vi "HEALTH_LABVIEW_V8.vi"() -> ()   [LabVIEW 2026]
uses:
  <vilib>/addons/control/pid/pid.llb/PID (DBL).vi
  <vilib>/addons/control/pid/NI_PID_pid.lvlib
panel:
  out "EXT SURF RTD HX SIDE":dbl format="%#_3g"
  out "BLOCK RTD HEATER SIDE":dbl format="%#_3g"
  out "BLOCK RTD HX SIDE":dbl format="%#_3g"
  out "EXT SURF RTD HEATER SIDE":dbl format="%#_3g"
  out "COPPER BLOCK RTDs":cluster{dbl, dbl, dbl, dbl}(graph)
  in  "CLEAR GRAPHS":bool
  in  "PUMP PID GAINS":T1={"proportional gain (Kc)"=1.0, "integral time (Ti, min)"=0.01, "derivative time (Td, min)"=0.0} {"derivative time (Td, min)" format="%.3f"; "integral time (Ti, min)" format="%.3f"; "proportional gain (Kc)" format="%.3f"}
  in  "TARGET FLOW RATE (LPM)":dbl format="%.2f"
  out "OUTLET TEMP (C)":dbl format="%#_3g"
  out "INLET TEMP (C)":dbl format="%#_3g"
  out "PRESSURE DROP (PSI)":dbl(graph)
  out "DELTA T (C)":dbl format="%#_3f"
  out "DELTA T (C)":dbl(graph)
  out "COOLANT FLOW RATE":dbl(graph)
  in  "PUMP ON/OFF":bool
  in  "HEATER ON/OFF":bool
  in  "stop":bool
  out "Error String":string
  out "error out":errorcluster
  out "ConnectionType Out":i32
  out "DeviceType Out":i32
  in  "Identifier":string="LJM_idANY"
  in  "ConnectionType":string="LJM_ctANY"
  in  "DeviceType":string="LJM_dtANY"
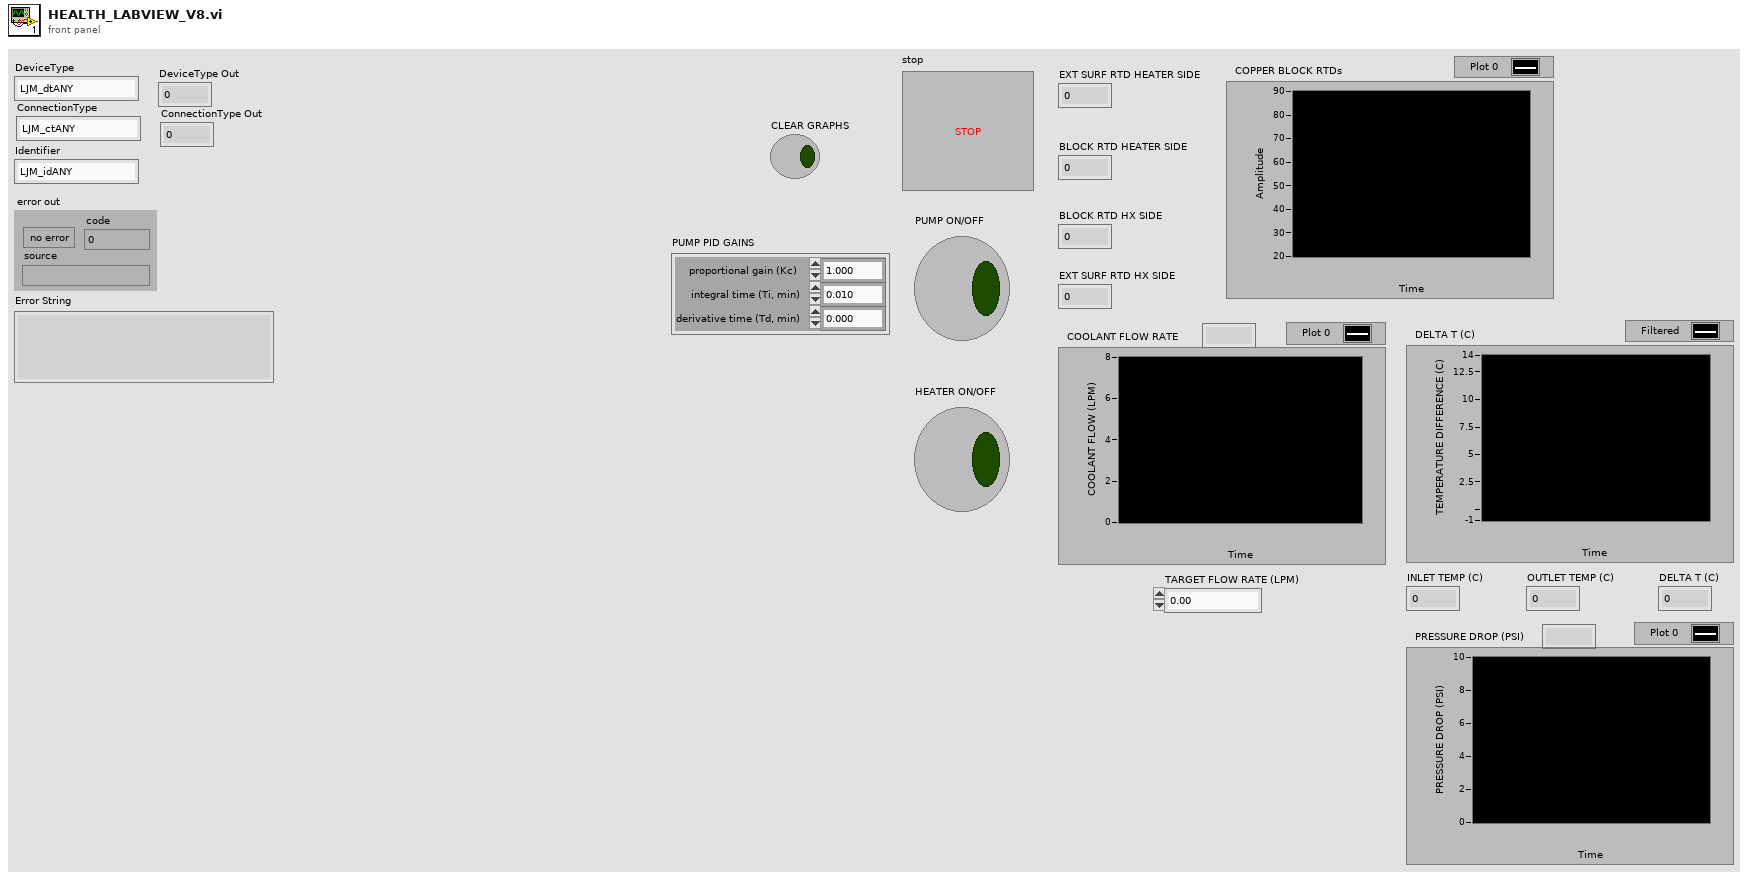
[diagram p1: front panel]
types:
  T1 = cluster{"proportional gain (Kc)":dbl, "integral time (Ti, min)":dbl, "derivative time (Td, min)":dbl}
  T2 = cluster{"dx/dt":dbl, "dx/dt":dbl, "dx/dt":dbl, "dx/dt":dbl, "dx/dt":dbl, "dx/dt":dbl}[]
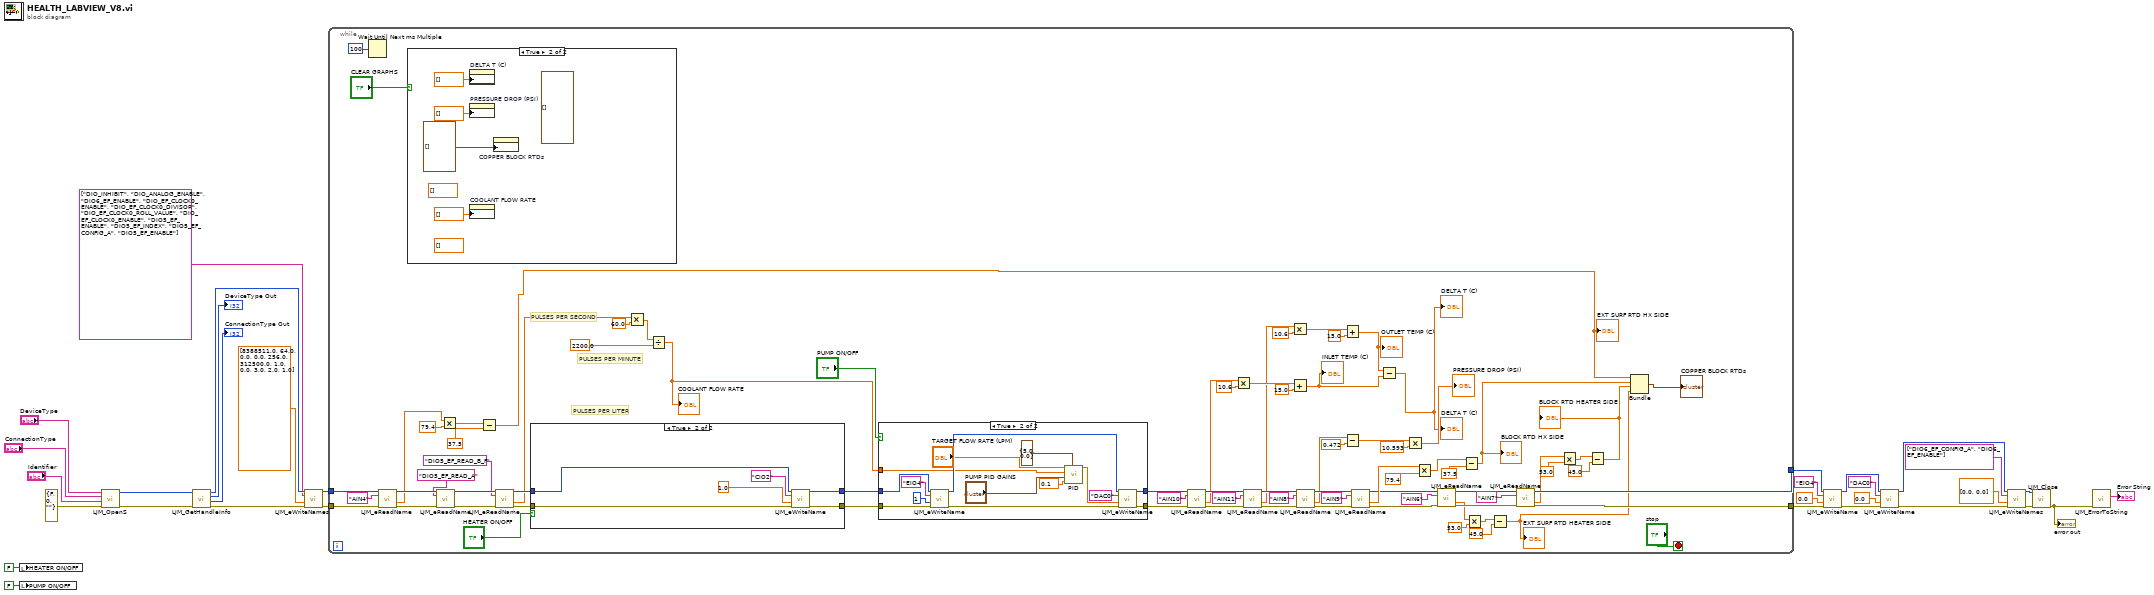
[diagram p0: block diagram]
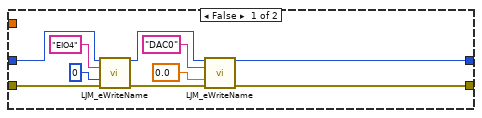
[diagram p3: hidden frame]
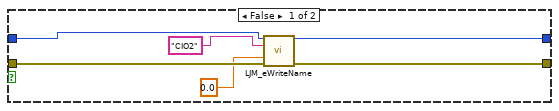
[diagram p4: hidden frame]
diagram:
  n1 = local write "HEATER ON/OFF"(FALSE ("HEATER ON/OFF 2")) -> ()
  n2 = local write "PUMP ON/OFF"(FALSE ("PUMP ON/OFF 2")) -> ()
  n3 = call "LJM_OpenS.vi"("error in"=errorcluster {"status"=FALSE, "code"=0, "source"=""} ("error in (no error)"), "Identifier"="Identifier", "ConnectionType"="ConnectionType", "DeviceType"="DeviceType") -> ("error out"=w31:errorcluster, "Handle"=w30:i32)  [unwired: 6 in]
  n4 = call "LJM_GetHandleInfo.vi"("error in"=w31, "Handle In"=w30) -> ("error out"=w21:errorcluster, "ConnectionType"=→"ConnectionType Out":i32, "DeviceType"=→"DeviceType Out":i32, "Handle Out"=w22:i32)  [unwired: 2 in, 4 out]
  n5 = call "LJM_eWriteNames.vi"("Handle In"=w22, "aNames"=string[] ["DIO_INHIBIT", "DIO_ANALOG_ENABLE", "DIO6_EF_ENABLE", "DIO_EF_CLOCK0_ENABLE", "DIO_EF_CLOCK0_DIVISOR", "DIO_EF_CLOCK0_ROLL_VALUE", "DIO_EF_CLOCK0_ENABLE", "DIO5_EF_ENABLE", "DIO5_EF_INDEX", "DIO5_EF_CONFIG_A", "DIO5_EF_ENABLE"], "aValuesIn"=dbl[] [8388511.0, 64.0, 0.0, 0.0, 256.0, 312500.0, 1.0, 0.0, 3.0, 2.0, 1.0], "error in"=w21) -> ("Handle Out"=w2:i32, "error out"=w1:errorcluster)  [unwired: 9 in, 1 out]
  n6 = while {
    tunnel: [w54] -> w9
    tunnel: w2 -> [w105]
    tunnel: w1 -> [w104]
    tunnel: [w53] -> w3
    stop <- "stop" stop-if-true
    # "PULSES PER LITER"
    # "PULSES PER MINUTE"
    # "PULSES PER SECOND"
    n7 = Wait Until Next ms Multiple(millisecond multiple=u32 100 ("milliseconds to wait")) -> ()  [unwired: 1 out]
    n8 = call "LJM_eReadName.vi"("Handle In"=w105, "Name"="AIN4", "error in"=w104) -> ("Handle Out"=w103:i32, "Value"=w63:dbl, "error out"=w102:errorcluster)  [unwired: 10 in]
    n9 = case shown="True" "CLEAR GRAPHS" {
      frame False {
      }
      frame True {
        (unwired) T2 [] ("History Data")
        (unwired) dbl[] [] ("History Data")
        (unwired) dbl[] [] ("History Data")
        n10 = property on="DELTA T (C)" class="WFChart (strict)"("History Data"=dbl[] []) -> ()  [unwired: 2 in, 2 out]
        n11 = property on="PRESSURE DROP (PSI)" class="WFChart (strict)"("History Data"=dbl[] []) -> ()  [unwired: 2 in, 2 out]
        n12 = property on="COOLANT FLOW RATE" class="WFChart (strict)"("History Data"=dbl[] []) -> ()  [unwired: 2 in, 2 out]
        n13 = property on="COPPER BLOCK RTDs" class="WFChart (strict)"("History Data"=cluster{dbl, dbl, dbl, dbl}[] []) -> ()  [unwired: 2 in, 2 out]
      }
    }
    n14 = call "LJM_eReadName.vi"("Handle In"=w103, "Name"="DIO5_EF_READ_A", "error in"=w102) -> ("Handle Out"=w100:i32, "error out"=w97:errorcluster)  [unwired: 10 in, 1 out]
    n15 = Multiply(x=w63, y=79.4 ("Address 2")) -> (x*y=w62:dbl)
    n16 = Subtract(x=w62, y=37.5) -> (x-y=w34:dbl)
    "EXT SURF RTD HX SIDE" <- w34
    n17 = call "LJM_eReadName.vi"("Handle In"=w100, "Name"="DIO5_EF_READ_B_F" ("DIO5_EF_READ_B_F"), "error in"=w97) -> ("Handle Out"=w99:i32, "Value"=w72:dbl, "error out"=w98:errorcluster)  [unwired: 10 in]
    n18 = case shown="True" "HEATER ON/OFF" {
      tunnel: [w146 w153] -> w106
      tunnel: [w147 w152] -> w107
      tunnel: w99 -> [w144 w150]
      tunnel: w98 -> [w143 w149]
      frame False {
        n19 = call "LJM_eWriteName.vi"("Handle In"=w144, "Name"="CIO2", "Value"=0.0, "error in"=w143) -> ("Handle Out"=w147:i32, "error out"=w146:errorcluster)  [unwired: 10 in]
      }
      frame True {
        n20 = call "LJM_eWriteName.vi"("Handle In"=w150, "Name"="CIO2", "Value"=1.0, "error in"=w149) -> ("Handle Out"=w152:i32, "error out"=w153:errorcluster)  [unwired: 10 in]
      }
    }
    n21 = Multiply(x=w72, y=60.0) -> (x*y=w70:dbl)
    n22 = Divide(x=w70, y=2200.0) -> (x/y=w68:dbl)
    "COOLANT FLOW RATE" <- w68
    n23 = case shown="True" "PUMP ON/OFF" {
      tunnel: w107 -> [w124 w139]
      tunnel: w106 -> [w123 w138]
      tunnel: [w119 w133] -> w91
      tunnel: [w118 w134] -> w95
      tunnel: w68 -> [_ w132]
      frame False {
        n24 = call "LJM_eWriteName.vi"("Handle In"=w124, "Name"="EIO4", "Value"=0, "error in"=w123) -> ("Handle Out"=w121:i32, "error out"=w120:errorcluster)  [unwired: 10 in]
        n25 = call "LJM_eWriteName.vi"("Handle In"=w121, "Name"="DAC0", "Value"=0.0, "error in"=w120) -> ("Handle Out"=w118:i32, "error out"=w119:errorcluster)  [unwired: 10 in]
      }
      frame True {
        n26 = call "LJM_eWriteName.vi"("Handle In"=w139, "Name"="EIO4", "Value"=1, "error in"=w138) -> ("Handle Out"=w135:i32, "error out"=w136:errorcluster)  [unwired: 10 in]
        n27 = call-poly <vilib>:"PID.vi"("output range"=cluster{"output high":dbl, "output low":dbl} {"output high"=5.0, "output low"=0.0}, "dt (s)"=0.1 ("FLOW dt (s)"), "PID gains"="PUMP PID GAINS", "process variable"=w132, "setpoint"="TARGET FLOW RATE (LPM)") -> ("output"=w127:dbl)  [unwired: 5 in, 1 out]
        n28 = call "LJM_eWriteName.vi"("Handle In"=w135, "Name"="DAC0", "Value"=w127, "error in"=w136) -> ("Handle Out"=w134:i32, "error out"=w133:errorcluster)  [unwired: 10 in]
      }
    }
    n29 = call "LJM_eReadName.vi"("Handle In"=w95, "Name"="AIN10", "error in"=w91) -> ("Handle Out"=w94:i32, "Value"=w66:dbl, "error out"=w90:errorcluster)  [unwired: 10 in]
    n30 = Multiply(x=w66, y=10.6) -> (x*y=w82:dbl)
    n31 = call "LJM_eReadName.vi"("Handle In"=w94, "Name"="AIN11" ("Name 2"), "error in"=w90) -> ("Handle Out"=w93:i32, "Value"=w65:dbl, "error out"=w89:errorcluster)  [unwired: 10 in]
    n32 = Multiply(x=w65, y=10.6) -> (x*y=w79:dbl)
    n33 = Add(x=w82, y=15.0) -> (x+y=w38:dbl)
    "INLET TEMP (C)" <- w38
    n34 = call "LJM_eReadName.vi"("Handle In"=w93, "Name"="AIN8" ("Name 3"), "error in"=w89) -> ("Handle Out"=w92:i32, "Value"=w73:dbl, "error out"=w88:errorcluster)  [unwired: 10 in]
    n35 = Add(x=w79, y=15.0) -> (x+y=w37:dbl)
    "OUTLET TEMP (C)" <- w37
    n36 = Subtract(x=w73, y=0.472) -> (x-y=w76:dbl)
    n37 = call "LJM_eReadName.vi"("Handle In"=w92, "Name"="AIN9" ("Name 4"), "error in"=w88) -> ("Handle Out"=w56:i32, "Value"=w60:dbl, "error out"=w51:errorcluster)  [unwired: 10 in]
    n38 = Subtract(x=w37, y=w38) -> (x-y=→"DELTA T (C)" →"DELTA T (C)":dbl)
    n39 = Multiply(x=w76, y=10.593) -> (x*y=→"PRESSURE DROP (PSI)":dbl)
    n40 = Multiply(x=w60, y=79.4) -> (x*y=w58:dbl)
    n41 = call "LJM_eReadName.vi"("Handle In"=w56, "Name"="AIN6", "error in"=w51) -> ("Handle Out"=w55:i32, "Value"=w47:dbl, "error out"=w52:errorcluster)  [unwired: 10 in]
    n42 = Subtract(x=w58, y=37.5) -> (x-y=w36:dbl)
    "BLOCK RTD HX SIDE" <- w36
    n43 = Multiply(x=w47, y=53.0) -> (x*y=w48:dbl)
    n44 = Subtract(x=w48, y=45.0) -> (x-y=w33:dbl)
    "EXT SURF RTD HEATER SIDE" <- w33
    n45 = call "LJM_eReadName.vi"("Handle In"=w55, "Name"="AIN7", "error in"=w52) -> ("Handle Out"=w54:i32, "Value"=w42:dbl, "error out"=w53:errorcluster)  [unwired: 10 in]
    n46 = Multiply(x=w42, y=53.0) -> (x*y=w44:dbl)
    n47 = Subtract(x=w44, y=45.0) -> (x-y=w35:dbl)
    "BLOCK RTD HEATER SIDE" <- w35
    n48 = Bundle(w34, w36, w35, w33) -> (→"COPPER BLOCK RTDs":cluster{dbl, dbl, dbl, dbl})  [unwired: 1 in]
  }
  n49 = call "LJM_eWriteName.vi"("Handle In"=w9, "Name"="EIO4", "Value"=0.0, "error in"=w3) -> ("Handle Out"=w10:i32, "error out"=w13:errorcluster)  [unwired: 10 in]
  n50 = call "LJM_eWriteName.vi"("Handle In"=w10, "Name"="DAC0", "Value"=0.0, "error in"=w13) -> ("Handle Out"=w11:i32, "error out"=w12:errorcluster)  [unwired: 10 in]
  n51 = call "LJM_eWriteNames.vi"("Handle In"=w11, "aNames"=string[] ["DIO6_EF_CONFIG_A", "DIO6_EF_ENABLE"], "aValuesIn"=dbl[] [0.0, 0.0], "error in"=w12) -> ("Handle Out"=w17:i32, "error out"=w18:errorcluster)  [unwired: 9 in, 1 out]
  n52 = call "LJM_Close.vi"("error in"=w18, "Handle"=w17) -> ("error out"=w23:errorcluster)  [unwired: 9 in]
  "error out" <- w23
  n53 = call "LJM_ErrorToString.vi"("error in"=w23) -> ("String"=→"Error String":string)  [unwired: 10 in]
